vi "Scratch_01.vi"() -> ()   [LabVIEW 2026]
panel:
  out "Numeric 2":i32
  out "Numeric":i32
  out "Shift Register result":i32
  out "Tunnel result":i32
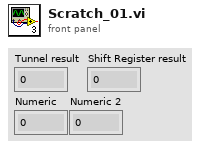
[diagram p1: front panel]
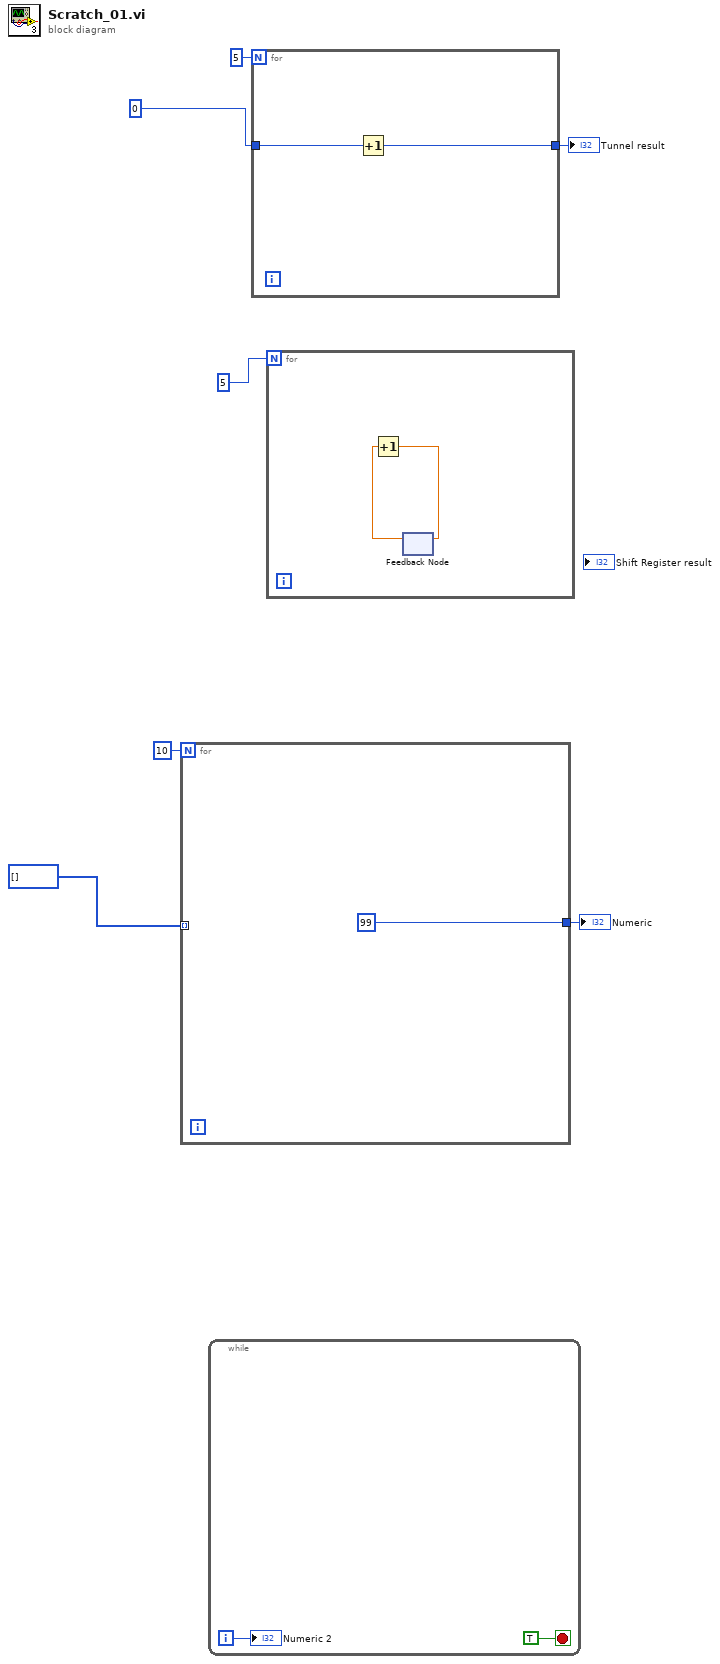
[diagram p0: block diagram]
diagram:
  n1 = for {
    N: 10 -> [_]
    tunnel: [99] -> w2
    tunnel: i32[] [] -> [_] mode=indexing
  }
  "Numeric" <- w2
  n2 = while {
    i -> [w9]
    stop <- TRUE stop-if-true
    "Numeric 2" <- w9
  }
  n3 = for {
    N: 5 -> [_]
    tunnel: 0 -> [w12]
    tunnel: [w11] -> w6
    n4 = Increment(x=w12) -> (x+1=w11:i32)
  }
  "Tunnel result" <- w6
  n5 = for {
    N: 5 -> [_]
    n6 = feedback #1() -> (w14:dbl)  [unwired: 1 in]
    n7 = Increment(x=w14) -> (x+1=w13:dbl)
    n8 = feedback-in #1(w13) -> ()
  }
